vi "MainLUTQualifiedNameParser.vi"(10 "Sample Number":u32, 11 "Run ID":string) -> (3 "QualifiedName":string)   [LabVIEW 2026]
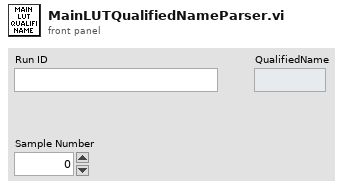
[diagram p1: front panel]
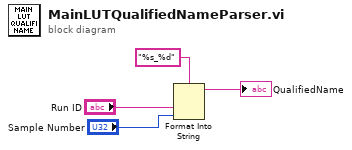
[diagram p0: block diagram]
diagram:
  n1 = Format Into String(format string="%s_%d", "Run ID", "Sample Number") -> (resulting string=→"QualifiedName":string)  [unwired: 2 in, 1 out]
